vi "ADV Compute.vi"(8 "error in":errorcluster, 10 "ADV String":string, 11 "Water Tunnel Results in":refnum<class "Water Tunnel Results.lvclass">) -> (0 "error out":errorcluster, 2 "ADV":T1, 3 "Water Tunnel Results out":refnum<class "Water Tunnel Results.lvclass">)   [LabVIEW 2019, in "Results.lvlib" / "Water Tunnel Results.lvclass"]
uses:
  Water Tunnel Results.lvclass
  Water Tunnel Results.lvclass/Water Tunnel Results.ctl
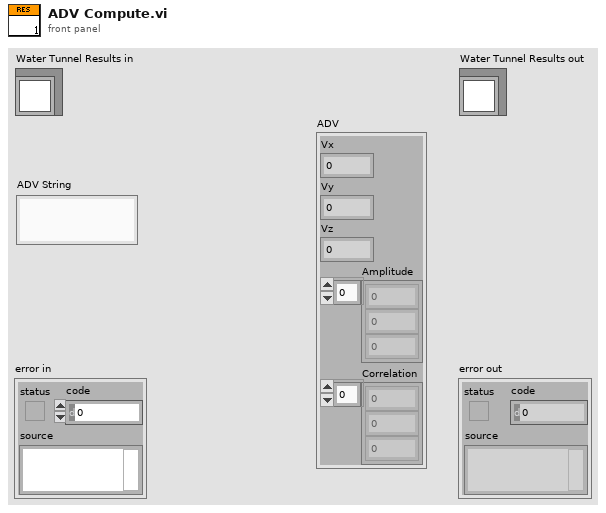
[diagram p1: front panel]
types:
  T1 = cluster{"Vx":dbl, "Vy":dbl, "Vz":dbl, "Amplitude":dbl[], "Correlation":dbl[]}
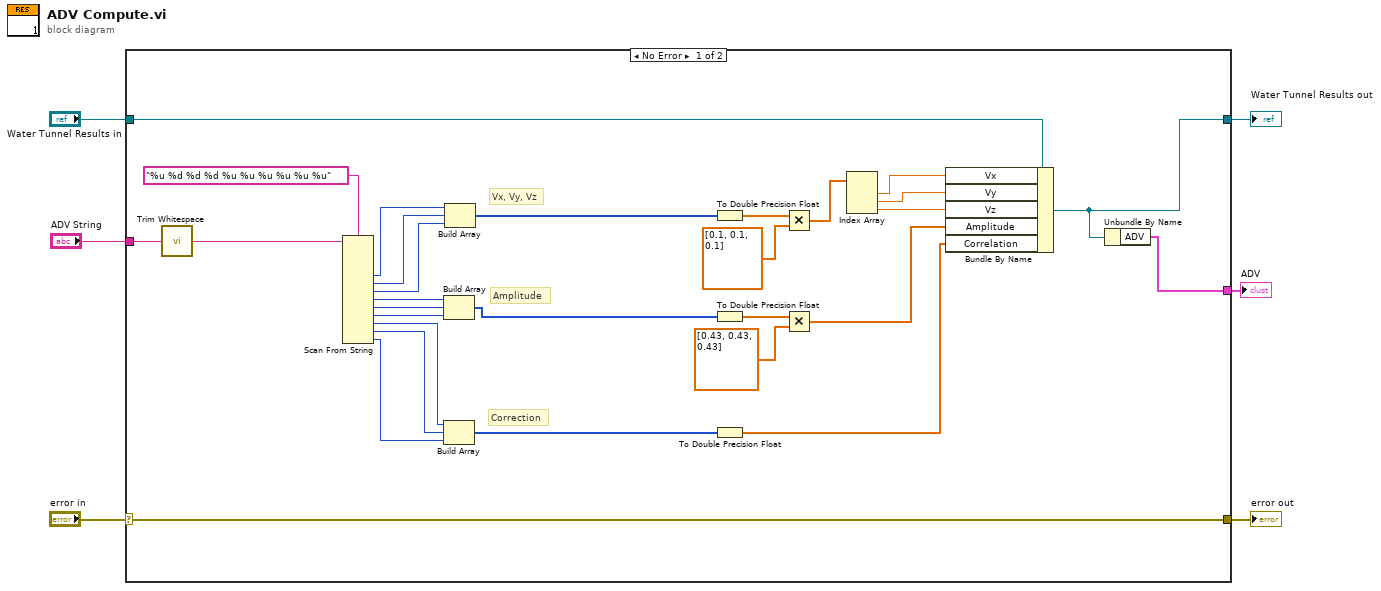
[diagram p0: block diagram]
diagram:
  n1 = case shown="No Error" "error in" {
    selector: "error in" -> [w35 w37]
    tunnel: [w35 w37] -> w5
    tunnel: [w27 w36] -> w3
    tunnel: "Water Tunnel Results in" -> [w34 w36]
    tunnel: "ADV String" -> [w21 _]
    tunnel: [w26 _] -> w1
    frame No Error {
      # "Correction"
      # "Amplitude"
      # "Vx, Vy, Vz"
      n2 = call <vilib>:"Trim Whitespace.vi"("string"=w21) -> ("trimmed string"=w20:string)  [unwired: 1 in]
      n3 = Scan From String(format string="%u %d %d %d %u %u %u %u %u %u", input string=w20) -> (output 2=w18:i32, output 3=w17:i32, output 4=w16:i32, output 5=w14:u32, output 6=w13:u32, output 7=w12:u32, output 8=w10:u32, output 9=w9:u32, output 10=w8:u32)  [unwired: 13 in, 3 out]
      n4 = Build Array(w14, w13, w12) -> (w11:u32[])
      n5 = Build Array(w10, w9, w8) -> (w7:u32[])
      n6 = Build Array(w18, w17, w16) -> (w15:i32[])
      n7 = To Double Precision Float(number=w15) -> (double precision float=w33:dbl[])
      n8 = To Double Precision Float(number=w11) -> (double precision float=w24:dbl[])
      n9 = To Double Precision Float(number=w7) -> (double precision float=w23:dbl[])
      n10 = Multiply(x=w33, y=dbl[] [0.1, 0.1, 0.1]) -> (x*y=w31:dbl[])
      n11 = Multiply(x=w24, y=dbl[] [0.43, 0.43, 0.43]) -> (x*y=w22:dbl[])
      n12 = Index Array(array=w31) -> (element #1=w30:dbl, element #2=w29:dbl, element #3=w28:dbl)  [unwired: 3 in]
      n13 = Bundle By Name(cluster=w34, "Vx"=w30, "Vy"=w29, "Vz"=w28, "Amplitude"=w22, "Correlation"=w23) -> (w27:refnum<class "Water Tunnel Results.lvclass">)
      n14 = Unbundle By Name(w27) -> ("ADV"=w26:T1)
    }
    frame Error {
    }
  }
  "error out" <- w5
  "Water Tunnel Results out" <- w3
  "ADV" <- w1
